vi "VIH - CHM Project - Write IDX File - Add IDX Record.vi"(6 "Level":i32, 7 "Base Dir Path":path, 9 "Topics":cluster{"HTML Path":path, "HTML Title":string}[](array[cluster]), 10 "Keyword":string, 11 "HTML in":string) -> (3 "HTML out":string)   [LabVIEW 2014]
doc: "::: VI Helpeks :::\nCopyright (c) 2000-2026 Konstantin Shifershteyn. All rights reserved."
panel:
  # "VI Helpeks\nCopyright (c) 2012-2026 Konstantin Shifershteyn"
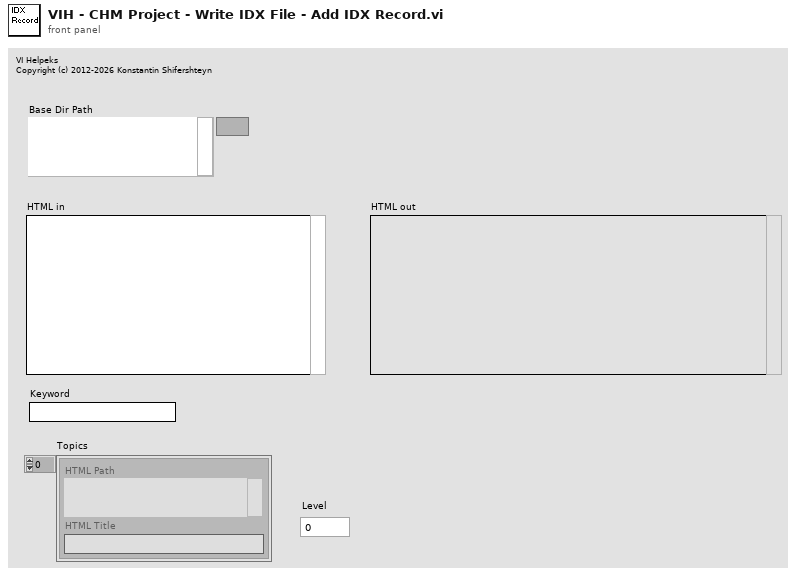
[diagram p1: front panel]
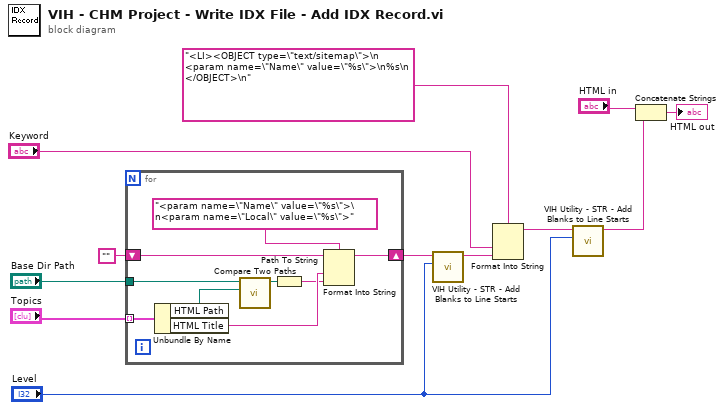
[diagram p0: block diagram]
diagram:
  n1 = for {
    tunnel: "Topics" -> [w21] mode=indexing
    tunnel: "Base Dir Path" -> [w16]
    shift-right: [w14] -> w3
    shift-left: "" -> [w13]
    n2 = Unbundle By Name(w21) -> ("HTML Path"=w18:path, "HTML Title"=w19:string)
    n3 = call <vilib>:"Compare Two Paths.vi"("Path 2"=w18, "Path 1"=w16) -> ("Relative Path from 1 to 2"=w20:path)  [unwired: 6 in, 3 out]
    n4 = Path To String(path=w20) -> (string=w17:string)
    n5 = Format Into String(format string="<param name=\"Name\" value=\"%s\">\n<param name=\"Local\" value=\"%s\">", initial string=w13, w19, w17) -> (resulting string=w14:string)  [unwired: 1 in, 1 out]
  }
  n6 = call "VIH Utility - STR - Add Blanks to Line Starts.vi"("level"="Level", "String"=w3) -> ("String out"=w2:string)  [unwired: 9 in]
  n7 = Format Into String(format string="<LI><OBJECT type=\"text/sitemap\">\n  <param name=\"Name\" value=\"%s\">\n%s\n  </OBJECT>\n", "Keyword", w2) -> (resulting string=w6:string)  [unwired: 2 in, 1 out]
  n8 = call "VIH Utility - STR - Add Blanks to Line Starts.vi"("level"="Level", "String"=w6) -> ("String out"=w10:string)  [unwired: 9 in]
  n9 = Concatenate Strings("HTML in", w10) -> (→"HTML out":string)
